vi "MQTT Data - Decode Varint.vi"(7 "Variable Length Integer Data":u8[](array[numeric])) -> (4 "remaining data":u8[](array[numeric]), 8 "Value":i32, 10 "Size (bytes)":i32)   [LabVIEW 2019, in "KoRE-MQTT.lvlib"]
doc: "Copyright (c) 2025 KoRElibs.com\nSPDX-License-Identifier: EUPL-1.2\n\nThis VI is licensed under the European Union Public License (EUPL) Version 1.2. You may use this VI unmodified in proprietary works. If you distribute a modified version of this file, the modified file must be released under the EUPL-1.2. Full license: https://joinup.ec.europa.eu/asset/eupl/eupl/1.2/"
uses:
  KoRE-MQTT.lvlib
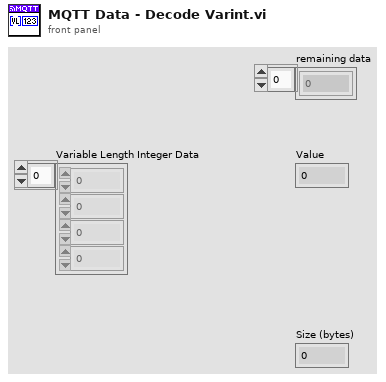
[diagram p1: front panel]
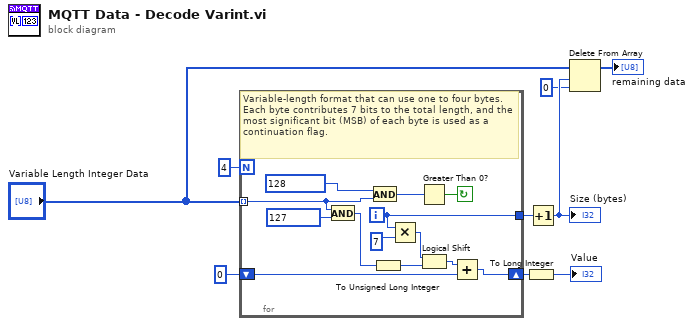
[diagram p0: block diagram]
diagram:
  n1 = for {
    N: 4 -> [_]
    tunnel: "Variable Length Integer Data" -> [w21] mode=indexing
    shift-right: [w15] -> w6
    shift-left: u32 0 -> [w14]
    tunnel: [w10] -> w7
    i -> [w10]
    stop <- w18 continue-if-true
    # "Variable-length format that can use one to four bytes. Each byte contributes 7 bits to the total length, and the most significant bit (MSB) of each byte is used as a continuation flag."
    n2 = And(x=w21, y=u8 127) -> (x .and. y?=w17:u8)
    n3 = And(x=u8 128, y=w21) -> (x .and. y?=w19:u8)
    n4 = To Unsigned Long Integer(number=w17) -> (unsigned 32bit integer=w13:u32)
    n5 = Multiply(x=w10, y=7) -> (x*y=w16:i32)
    n6 = Greater Than 0?(x=w19) -> (x > 0?=w18:bool)
    n7 = Logical Shift(y=w16, x=w13) -> (x << y=w12:u32)
    n8 = Add(x=w12, y=w14) -> (x+y=w15:u32)
  }
  n9 = To Long Integer(number=w6) -> (32bit integer=→"Value":i32)
  n10 = Increment(x=w7) -> (x+1=w3:i32)
  "Size (bytes)" <- w3
  n11 = Delete From Array(array="Variable Length Integer Data", length=w3, index=0) -> (array with subset deleted=→"remaining data":u8[])  [unwired: 1 out]
